vi "VIH ExtCmd - Associate VIHRUN.vi"(8 "error in":errorcluster) -> (0 "error out":errorcluster)   [LabVIEW 2014]
doc: "::: VI Helpeks :::\nCopyright (c) 2000-2026 Konstantin Shifershteyn. All rights reserved."
uses:
  <vilib>/registry/registry.llb/Registry RtKey.ctl
  <vilib>/registry/registry.llb/Registry SAM.ctl
  <vilib>/registry/registry.llb/Write Registry Value Simple STR.vi
panel:
  # "VI Helpeks\nCopyright (c) 2012-2026 Konstantin Shifershteyn"
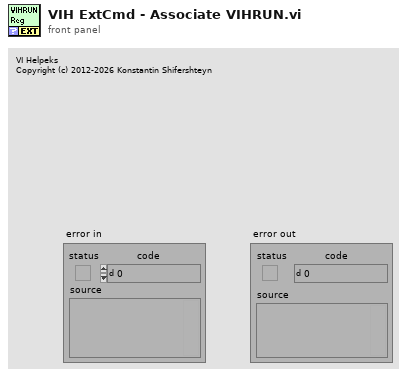
[diagram p1: front panel]
types:
  T1 = typedef "Registry SAM.ctl" = enum32{"KEY_QUERY_VALUE", "KEY_SET_VALUE", "KEY_CREATE_SUB_KEY", "KEY_ENUMERATE_SUB_KEYS", "KEY_NOTIFY", "KEY_CREATE_LINK", "KEY_READ", "KEY_WRITE", "KEY_ALL_ACCESS", "KEY_READ | KEY_WRITE"}
  T2 = typedef "Registry RtKey.ctl" = enum32{"HKEY_CLASSES_ROOT", "HKEY_CURRENT_USER", "HKEY_LOCAL_MACHINE", "HKEY_USERS", "HKEY_PERFORMANCE_DATA", "HKEY_CURRENT_CONFIG", "HKEY_DYN_DATA"}
  T3 = enum32{"REG_OPTION_NON_VOLATILE", "REG_OPTION_VOLATILE", "REG_OPTION_BACKUP_RESTORE"}
  T4 = cluster{"Product Name":string, "Short Name":string, "Product Version":string, "Release Timestamp":string, "Developer":string, "Copyright":string}
  T5 = cluster{"Extension":string, "Program ID":string, "DefaultIcon":string, "OpenCommand":string}
  T6 = typedef "Registry refnum.ctl" = refnum<k1>
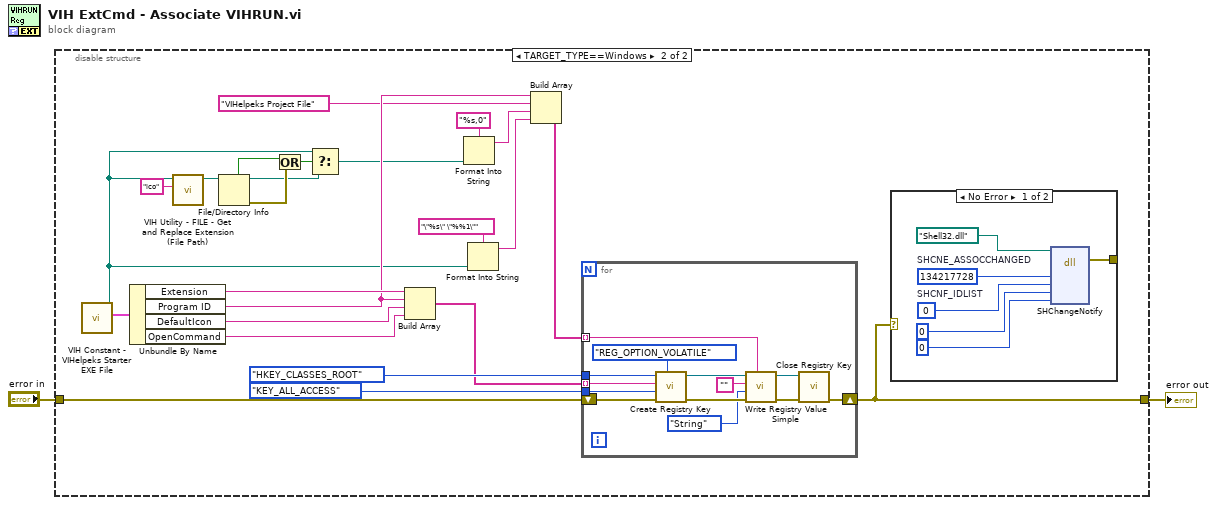
[diagram p0: block diagram]
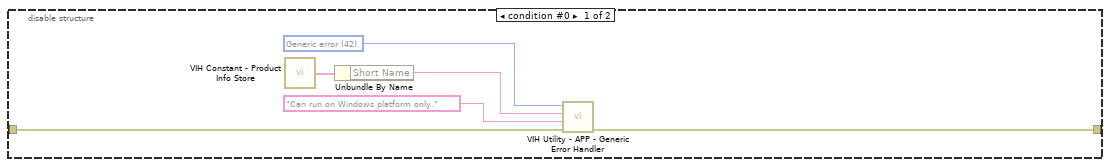
[diagram p2: hidden frame]
diagram:
  n1 = disable-structure shown="TARGET_TYPE==Windows" {
    disable-tunnel: "error in" -> [w4 w32]
    disable-tunnel: [w3 w31] -> w1
    frame condition #0 {
      w5 = 42 items=["No error", "Argument error", "Memory is full", "Out of zone", "End of file", "File already open", "Generic file I/O error", "File not found", "File permission error", "Disk is full", "Duplicate path", "Too many files open", "System feature not enabled", "Resource file not found", "Cannot add resource", "Resource not found", "Image not found", "Image memory error", "Pen does not exist", "Config type invalid", "Config token not found", "Config parse error", "Config memory error", "Bad external code format", "Bad external code offset", "External code not present", "Null window", "Destroy window error", "Null menu", "Print aborted", "Bad print record", "Print driver error", "Windows error during printing", "Memory error during printing", "Print dialog error", "Generic print error", "Invalid device refnum", "Device not found", "Device parameter error", "Device unit error", "Cannot open device", "Device call aborted", "Generic error", "Cancelled by user", "Object ID too low", "Object ID too high", "Object not in heap", "Unknown heap", "Unknown object (invalid DefProc)", "Unknown object (DefProc not in table)", "Message out of range", "Invalid (null) method", "Unknown message", "Manager call not supported", "Bad address", "Network operation in progress", "Network operation timed out", "Connection is busy", "Network attribute not supported", "Network error", "Address in use", "System out of memory", "Connection aborted", "Connection refused", "Not connected", "Already connected", "Connection closed", "Initialization error (interapplication manager)", "Bad occurrence", "Wait on unbound occurrence handler", "Occurrence queue overflow", "Datalog type conflict", "Unused", "Unrecognized type (interapplication manager)", "Memory corrupt", "Failed to make temporary DLL", "Old CIN version", "Drag socket not found", "Failed to load drop-object", "Failed to register OLE object", "Failed to release OLE object", "Format specifier type mismatch", "Unknown format specifier", "Too few format specifiers", "Too many format specifiers", "Scan failed", "Newer CIN version", "Error converting to variant", "Runtime menu error", "Password tampered", "Variant attribute not found", "Incompatible variant data type", "Event data is not available", "Event Store is not present", "Occurrence is not found", "Event Queue is not created", "Event info is not available in the type library", "Refnum passed is NULL", "Error retrieving Class GUID", "Error retrieving CoClass GUID", "Error retrieving TypeLib GUID.", "Bad built application magic bytes.", "Specific driver is different from the specific driver associated with the Logical Name.", "There is no session opened to the class driver.", "Max Error", "MAX - Error with config objects", "MAX - Error loading configuration", "MAX - Group not supported", "Singlecast connections can not send to multicast addresses.", "Multicast connections can not send to singlecast addresses.", "Specified IP address not in multicast address range.", "Attempt to write to read-only multicast connection.", "Attempt to read from write-only multicast connection.", "The buffer used to receive a datagram was smaller than the datagram itself"]
      n2 = call "VIH Constant - Product Info Store.vi"() -> ("Product Info"=w7:T4)
      n3 = Unbundle By Name(w7) -> ("Short Name"=w8:string)
      n4 = call "VIH Utility - APP - Generic Error Handler.vi"("error in"=w4, "error reason"="Can run on Windows platform only.", "error location"=w8, "error code"=w5) -> ("error out"=w3:errorcluster)  [unwired: 6 in, 1 out]
    }
    frame condition #1 (active) {
      n5 = call "VIH Constant - VIHelpeks Starter EXE File.vi"() -> ("Registry Keys"=w30:T5, "VIHelpeks Starter EXE path"=w10:path)  [unwired: 9 in, 1 out]
      n6 = Unbundle By Name(w30) -> ("Extension"=w27:string, "Program ID"=w23:string, "DefaultIcon"=w26:string, "OpenCommand"=w25:string)
      n7 = call "VIH Utility - FILE - Get and Replace Extension (File Path).vi"("new extension (none)"="ico", "file path"=w10) -> ("new file path"=w15:path)  [unwired: 8 in, 1 out]
      n8 = File/Directory Info(path=w15) -> (path out=w11:path, directory=w13:bool, error out=w14:errorcluster)  [unwired: 1 in, 4 out]
      n9 = Or(x=w13, y=w14) -> (x .or. y?=w12:bool)
      n10 = Select(t=w10, s=w12, f=w11) -> (s? t:f=w9:path)
      n11 = Build Array(w27, w23, w26, w25) -> (w24:string[])
      n12 = Format Into String(format string="%s,0", w9) -> (resulting string=w19:string)  [unwired: 2 in, 1 out]
      n13 = Format Into String(format string="\"%s\" \"%%1\"", w10) -> (resulting string=w18:string)  [unwired: 2 in, 1 out]
      n14 = Build Array(w23, "VIHelpeks Project File", w19, w18) -> (w17:string[])
      n15 = for {
        shift-right: [w41] -> w31
        shift-left: w32 -> [w51]
        tunnel: Registry_RtKey."HKEY_CLASSES_ROOT" ("root key (HKEY_LOCAL_MACHINE)") -> [w50]
        tunnel: Registry_SAM."KEY_ALL_ACCESS" ("security access mask (KEY_READ | KEY_WRITE)") -> [w49]
        tunnel: w24 -> [w46] mode=indexing
        tunnel: w17 -> [w40] mode=indexing
        n16 = call <vilib>:"Create Registry Key.vi"("options"=T3."REG_OPTION_VOLATILE", "error in (no error)"=w51, "security access mask (KEY_READ | KEY_WRITE)"=w49, "subkey"=w46, "root key (HKEY_LOCAL_MACHINE)"=w50) -> ("error out"=w47:errorcluster, "refnum out"=w48:T6)  [unwired: 4 in, 1 out]
        n17 = call-poly <vilib>:"Write Registry Value Simple.vi"("String/Binary data"=w40, "error in (no error)"=w47, "simple data type"=enum16{"String", "Binary", "DWORD"}."String", "value"="", "refnum"=w48) -> ("error out"=w43:errorcluster, "refnum out"=w42:T6)  [unwired: 3 in]
        n18 = call <vilib>:"Close Registry Key.vi"("error in (no error)"=w43, "refnum"=w42) -> ("error out"=w41:errorcluster)  [unwired: 5 in]
      }
      n19 = case shown="No Error" w31 {
        tunnel: [w33 _] -> _
        frame No Error {
          w35 = u32 134217728  # SHCNE_ASSOCCHANGED
          w36 = u16 0  # SHCNF_IDLIST
          n20 = dll-call lib="shell32.dll" fn="SHChangeNotify"(path in=path "Shell32.dll", "wEvent"=w35, "uFlags"=w36, "dwItem1"=u32 0, "dwItem2"=u32 0) -> (error out=w33:errorcluster)  [unwired: 7 in, 1 out]
        }
        frame Error {
        }
      }
    }
  }
  "error out" <- w1
